vi "OverlayCoordinateSystem.vi"(6 "Color":u32(colorbox)=16711680, 7 "GroupName":string, 8 "error in":errorcluster, 9 "Size":i32=50, 10 "ReferenceSystem":T1, 11 "Image Reference In":T3) -> (0 "error out":errorcluster, 3 "Image Reference Out":T3)   [LabVIEW 2020, in "OpenLvVision_Overlays.lvlib"]
doc: "Overlays the axis of an coordinate system."
uses:
  OpenLvVision_Overlays.lvlib
  <vilib>/OpenLvVision/OpenLvVision_Image/Management/TypeDef/OLV Image.ctl
  TypeDefs/ReferenceSystem.ctl
  TypeDefs/PointI32.ctl
  TypeDefs/Line.ctl
  TypeDefs/DrawingMode.ctl
  TypeDefs/Arrows.ctl
  <vilib>/OpenLvVision/OpenLvVision_Image/Management/OLV Management.lvlib
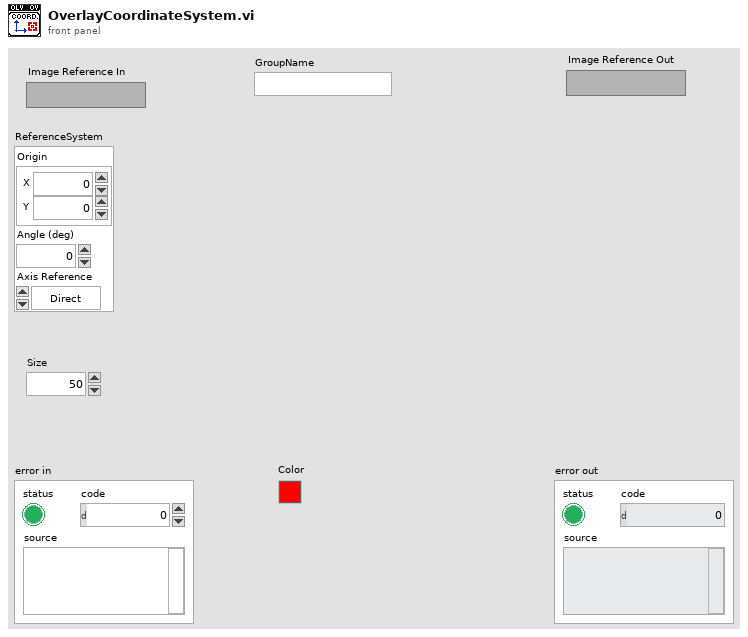
[diagram p1: front panel]
types:
  T1 = typedef "OpenLvVision_Overlays.lvlib/ReferenceSystem.ctl" = cluster{"Origin":T2, "Angle (deg)":dbl, "Axis Reference":enum16{"Direct", "Indirect"}}
  T2 = typedef "OpenLvVision_Overlays.lvlib/PointI32.ctl" = cluster{"X":i32, "Y":i32}
  T3 = typedef "OLV OpenLvVision_Image.lvlib/OLV Management.lvlib/OLV Image.ctl" = refnum<image>
  T4 = typedef "OpenLvVision_Overlays.lvlib/DrawingMode.ctl" = enum16{"Frame", "Fill"}
  T5 = cluster{"Desired Font (Application)":enum16{"User-specified Font", "Application Font", "System Font", "Dialog Font"}, "[User-specified Font]":cluster{"Font Name":string, "Size":i16, "Strikeout?":bool, "Italic?":bool, "Underline?":bool, "Outline?":bool, "Shadow?":bool, "Bold?":bool, "Rotation Angle":dbl}, "Horizontal Alignment":i16, "Vertical Alignment":i16}
  T6 = typedef "OpenLvVision_Overlays.lvlib/Line.ctl" = cluster{"StartPoint":T2, "EndPoint":T2}
  T7 = typedef "OpenLvVision_Overlays.lvlib/Arrows.ctl" = cluster{"StartPoint":bool, "StartArrowSize":dbl, "EndPoint":bool, "EndArrowSize":dbl}
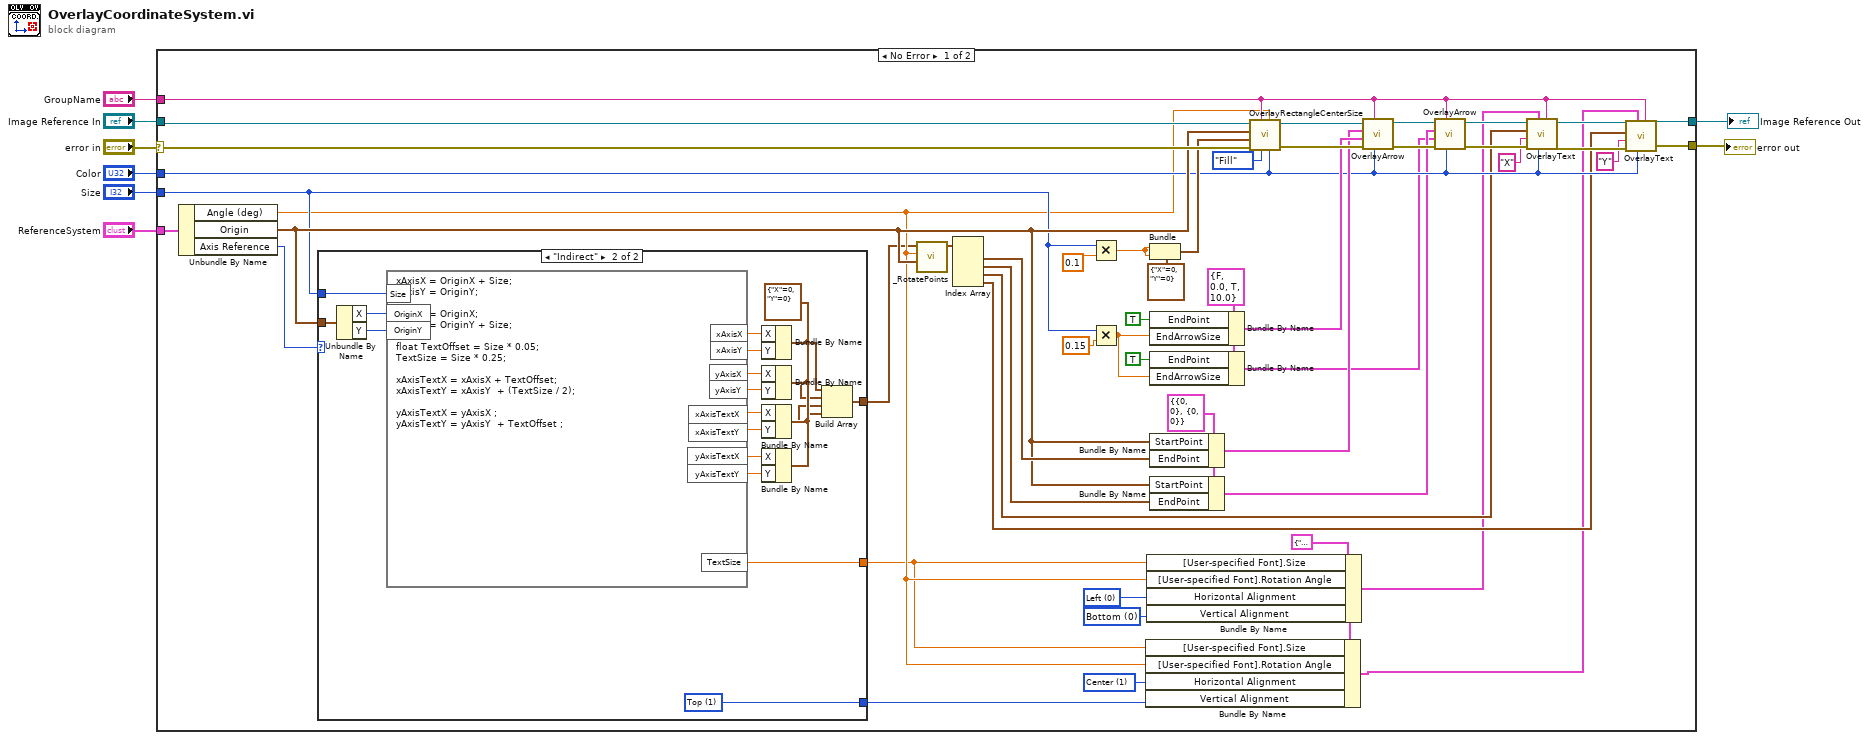
[diagram p0: block diagram]
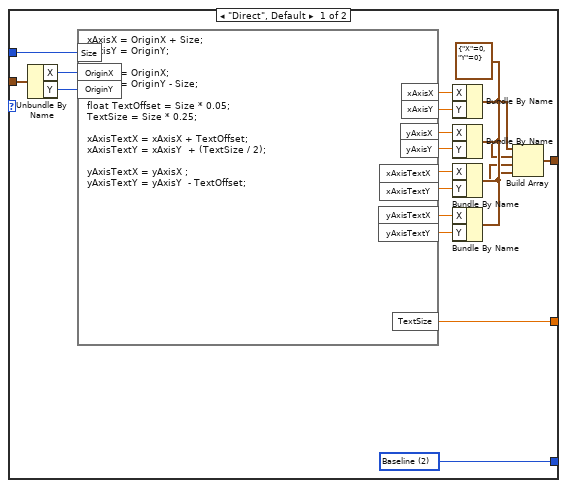
[diagram p2: hidden frame]
diagram:
  n1 = case shown="No Error" "error in" {
    selector: "error in" -> [w53 w99]
    tunnel: [w29 w99] -> w7
    tunnel: "Image Reference In" -> [w54 w100]
    tunnel: [w28 w100] -> w6
    tunnel: "Color" -> [w26 _]
    tunnel: "GroupName" -> [w27 _]
    tunnel: "ReferenceSystem" -> [w52 _]
    tunnel: "Size" -> [w20 _]
    frame No Error {
      w18 = i16 1 items=["Left", "Center", "Right"] ("Horizontal Alignment")
      w17 = i16 0 items=["Left", "Center", "Right"] ("Horizontal Alignment")
      w16 = i16 0 items=["Bottom", "Top", "Baseline"] ("Vertical Alignment")
      w14 = T5 {"Desired Font (Application)"=enum."User-specified Font", "[User-specified Font]"={"Font Name"="Application Font", "Size"=12, "Strikeout?"=FALSE, "Italic?"=FALSE, "Underline?"=FALSE, "Outline?"=FALSE, "Shadow?"=FALSE, "Bold?"=FALSE, "Rotation Angle"=0.0}, "Horizontal Alignment"=0, "Vertical Alignment"=0} ("Font, Size & Style")
      w41 = T6 {"StartPoint"={"X"=0, "Y"=0}, "EndPoint"={"X"=0, "Y"=0}} ("Line")
      w39 = T7 {"StartPoint"=FALSE, "StartArrowSize"=0.0, "EndPoint"=TRUE, "EndArrowSize"=10.0} ("Arrows")
      n2 = Unbundle By Name(w52) -> ("Angle (deg)"=w13:dbl, "Origin"=w34:T2, "Axis Reference"=w35:enum16{"Direct", "Indirect"})
      n3 = case shown="\"Indirect\"" w35 {
        tunnel: w34 -> [w77 w97]
        tunnel: w20 -> [w78 w98]
        tunnel: [w74 w94] -> w11
        tunnel: [w60 w80] -> w10
        tunnel: [w59 w79] -> w9
        frame "Direct", Default {
          w59 = i16 2 items=["Bottom", "Top", "Baseline"] ("Vertical Alignment")
          w69 = T2 {"X"=0, "Y"=0} ("Origin")
          n4 = Unbundle By Name(w77) -> ("X"=w76:i32, "Y"=w75:i32)
          n5 = formula code="xAxisX = OriginX + Size;\nxAxisY = OriginY;\n\nyAxisX = OriginX;\nyAxisY = OriginY - Size;\n\nfloat TextOffset = Size * 0.05;\nTextSize = Size * 0.25;\n\nxAxisTextX = xAxisX + TextOffset;\nxAxisTextY = xAxisY  + (TextSize / 2);\n\nyAxisTextX = yAxisX ;\nyAxisTextY = yAxisY  - TextOffset;"("Size"=w78, "OriginX"=w76, "OriginY"=w75) -> ("TextSize"=w74:dbl, "xAxisX"=w73:dbl, "xAxisY"=w72:dbl, "yAxisX"=w71:dbl, "yAxisY"=w70:dbl, "xAxisTextX"=w68:dbl, "xAxisTextY"=w67:dbl, "yAxisTextX"=w66:dbl, "yAxisTextY"=w65:dbl)
          n6 = Bundle By Name(cluster=w69, "X"=w73, "Y"=w72) -> (w61:T2)
          n7 = Bundle By Name(cluster=w69, "X"=w71, "Y"=w70) -> (w64:T2)
          n8 = Bundle By Name(cluster=w69, "X"=w68, "Y"=w67) -> (w63:T2)
          n9 = Bundle By Name(cluster=w69, "X"=w66, "Y"=w65) -> (w62:T2)
          n10 = Build Array(w61, w64, w63, w62) -> (w60:T2[])
        }
        frame "Indirect" {
          w79 = i16 1 items=["Bottom", "Top", "Baseline"] ("Vertical Alignment")
          w89 = T2 {"X"=0, "Y"=0} ("Origin")
          n11 = Unbundle By Name(w97) -> ("X"=w96:i32, "Y"=w95:i32)
          n12 = formula code="xAxisX = OriginX + Size;\nxAxisY = OriginY;\n\nyAxisX = OriginX;\nyAxisY = OriginY + Size;\n\nfloat TextOffset = Size * 0.05;\nTextSize = Size * 0.25;\n\nxAxisTextX = xAxisX + TextOffset;\nxAxisTextY = xAxisY  + (TextSize / 2);\n\nyAxisTextX = yAxisX ;\nyAxisTextY = yAxisY  + TextOffset ;"("Size"=w98, "OriginX"=w96, "OriginY"=w95) -> ("TextSize"=w94:dbl, "xAxisX"=w93:dbl, "xAxisY"=w92:dbl, "yAxisX"=w91:dbl, "yAxisY"=w90:dbl, "xAxisTextX"=w88:dbl, "xAxisTextY"=w87:dbl, "yAxisTextX"=w86:dbl, "yAxisTextY"=w85:dbl)
          n13 = Bundle By Name(cluster=w89, "X"=w93, "Y"=w92) -> (w81:T2)
          n14 = Bundle By Name(cluster=w89, "X"=w91, "Y"=w90) -> (w84:T2)
          n15 = Bundle By Name(cluster=w89, "X"=w88, "Y"=w87) -> (w83:T2)
          n16 = Bundle By Name(cluster=w89, "X"=w86, "Y"=w85) -> (w82:T2)
          n17 = Build Array(w81, w84, w83, w82) -> (w80:T2[])
        }
      }
      n18 = call "_RotatePoints.vi"("Origin"=w34, "Angle"=w13, "Points in"=w10) -> ("Points out"=w42:T2[])  [unwired: 8 in]
      n19 = Index Array(array=w42) -> (element #1=w37:T2, element #2=w36:T2, element #3=w25:T2, element #4=w24:T2)  [unwired: 4 in]
      n20 = Multiply(x=w20, y=0.1) -> (x*y=w46:dbl)
      n21 = Multiply(x=w20, y=0.15) -> (x*y=w43:dbl)
      n22 = Bundle By Name(cluster=w14, "[User-specified Font].Size"=w11, "[User-specified Font].Rotation Angle"=w13, "Horizontal Alignment"=w18, "Vertical Alignment"=w9) -> (w12:T5)
      n23 = Bundle By Name(cluster=w14, "[User-specified Font].Size"=w11, "[User-specified Font].Rotation Angle"=w13, "Horizontal Alignment"=w17, "Vertical Alignment"=w16) -> (w15:T5)
      n24 = Bundle(cluster=T2 {"X"=0, "Y"=0} ("Size"), "X"=w46, "Y"=w46) -> (w47:T2)
      n25 = Bundle By Name(cluster=w39, "EndPoint"=TRUE, "EndArrowSize"=w43) -> (w40:T7)
      n26 = Bundle By Name(cluster=w39, "EndPoint"=TRUE, "EndArrowSize"=w43) -> (w19:T7)
      n27 = Bundle By Name(cluster=w41, "StartPoint"=w34, "EndPoint"=w37) -> (w38:T6)
      n28 = Bundle By Name(cluster=w41, "StartPoint"=w34, "EndPoint"=w36) -> (w21:T6)
      n29 = call "OverlayRectangleCenterSize.vi"("Color"=w26, "Angle"=w13, "Drawing Mode (Frame)"=DrawingMode."Fill", "GroupName"=w27, "error in"=w53, "Size"=w47, "Center-Point"=w34, "Image Reference In"=w54) -> ("error out"=w55:errorcluster, "Image Reference Out"=w56:T3)  [unwired: 2 in]
      n30 = call "OverlayArrow.vi"("Color"=w26, "GroupName"=w27, "error in"=w55, "Arrows"=w40, "Line"=w38, "Image Reference In"=w56) -> ("error out"=w57:errorcluster, "Image Reference Out"=w58:T3)  [unwired: 4 in]
      n31 = call "OverlayArrow.vi"("Color"=w26, "GroupName"=w27, "error in"=w57, "Arrows"=w19, "Line"=w21, "Image Reference In"=w58) -> ("error out"=w32:errorcluster, "Image Reference Out"=w33:T3)  [unwired: 4 in]
      n32 = call "OverlayText.vi"("GroupName"=w27, "Text Color (black)"=w26, "Font, Size & Style"=w15, "error in"=w32, "Text"="X", "Origin"=w25, "Image Reference In"=w33) -> ("error out"=w30:errorcluster, "Image Reference Out"=w31:T3)  [unwired: 3 in]
      n33 = call "OverlayText.vi"("GroupName"=w27, "Text Color (black)"=w26, "Font, Size & Style"=w12, "error in"=w30, "Text"="Y", "Origin"=w24, "Image Reference In"=w31) -> ("error out"=w29:errorcluster, "Image Reference Out"=w28:T3)  [unwired: 3 in]
    }
    frame Error {
    }
  }
  "error out" <- w7
  "Image Reference Out" <- w6
